vi "Generate BitfilePath.vi"() -> (0 "Bitfile path":path)   [LabVIEW 2020, in "FPGA Addon DMA Channels Interleaved System Tests.lvclass"]
uses:
  FPGA Addon DMA Channels Interleaved System Tests.lvclass
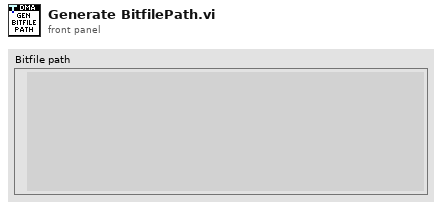
[diagram p1: front panel]
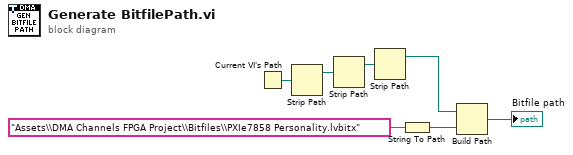
[diagram p0: block diagram]
diagram:
  n1 = Current VI's Path() -> (path=w6:path)
  n2 = Strip Path(path=w6) -> (stripped path=w5:path)  [unwired: 1 out]
  n3 = Strip Path(path=w5) -> (stripped path=w4:path)  [unwired: 1 out]
  n4 = Strip Path(path=w4) -> (stripped path=w2:path)  [unwired: 1 out]
  n5 = String To Path(string="Assets\\DMA Channels FPGA Project\\Bitfiles\\PXIe7858 Personality.lvbitx" ("name or relative path")) -> (path=w3:path)
  n6 = Build Path(base path=w2, name or relative path=w3) -> (appended path=→"Bitfile path":path)
